vi "Native_AddControl_v2.vi"() -> ()   [LabVIEW 2024]
panel:
  out "error out":errorcluster caption="错误输出"
  out "terminal_id":u32
  in  "terminal_id type":u32
  out "object_id":u32
  in  "object_id type":u32
  in  "label":string
  in  "y":i16=100
  in  "x":i16=100
  in  "style":u32
  in  "target_path":path
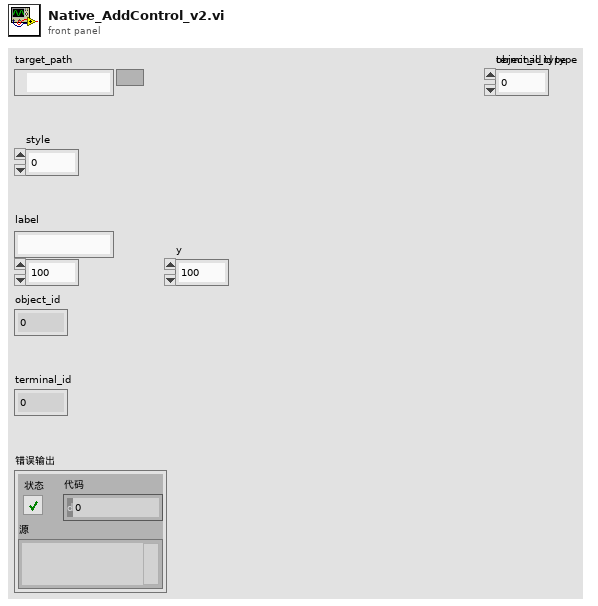
[diagram p1: front panel]
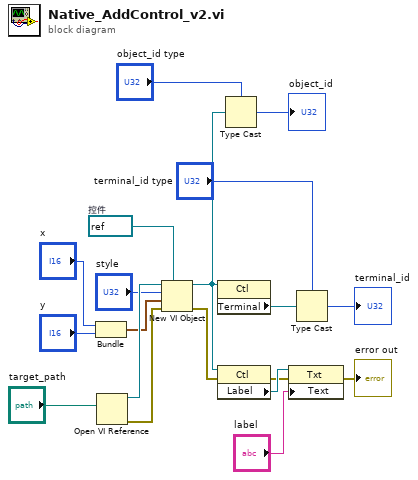
[diagram p0: block diagram]
diagram:
  w18 = refnum<vi> refnum  # 控件
  n1 = Bundle ("捆绑")("x"="x", "y"="y") -> (w12:cluster{"x":i16, "y":i16})  [unwired: 1 in]
  n2 = Open VI Reference ("打开VI引用")(vi path="target_path") -> (vi reference=w17:refnum<vi>, error out=w16:errorcluster)  [unwired: 5 in]
  n3 = New VI Object ("新建VI对象")(vi object class=w18, owner refnum=w17, style="style", position/next to=w12, 8:w16) -> (object refnum=w11:refnum<vi>, 0:w8:errorcluster)  [unwired: 3 in]
  n4 = property on="属性节点" class="Ctl"(reference=w11) -> ("Terminal"=w4:refnum<vi>)  [unwired: 1 in, 2 out]
  n5 = property on="属性节点" class="Ctl"(reference=w11, error in=w8) -> (error out=w7:errorcluster, "Label"=w10:refnum<vi>)  [unwired: 1 out]
  n6 = Type Cast ("强制类型转换")(type="object_id type", x=w11) -> (*(type *) &x=→"object_id":u32)
  n7 = property on="属性节点" class="Txt"(reference=w10, error in=w7, "Text"="label") -> (error out=→"error out":errorcluster)  [unwired: 1 out]
  n8 = Type Cast ("强制类型转换")(type="terminal_id type", x=w4) -> (*(type *) &x=→"terminal_id":u32)
